vi "Generer_listing.vi"(1 "Listing_entrée":string, 2 "Numéro de programme":u8, 3 "Programme":cluster{"chaîne":string, "Valeur":dbl}[][](array[cluster]) {"Valeur" format="%#.1f"}) -> (0 "Listing_sortie":string)   [LabVIEW 2022 SP3]
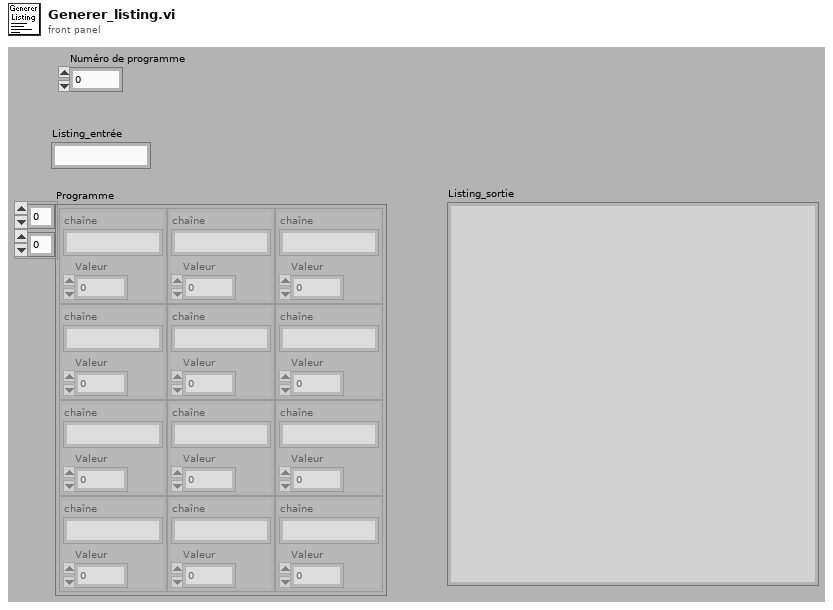
[diagram p1: front panel]
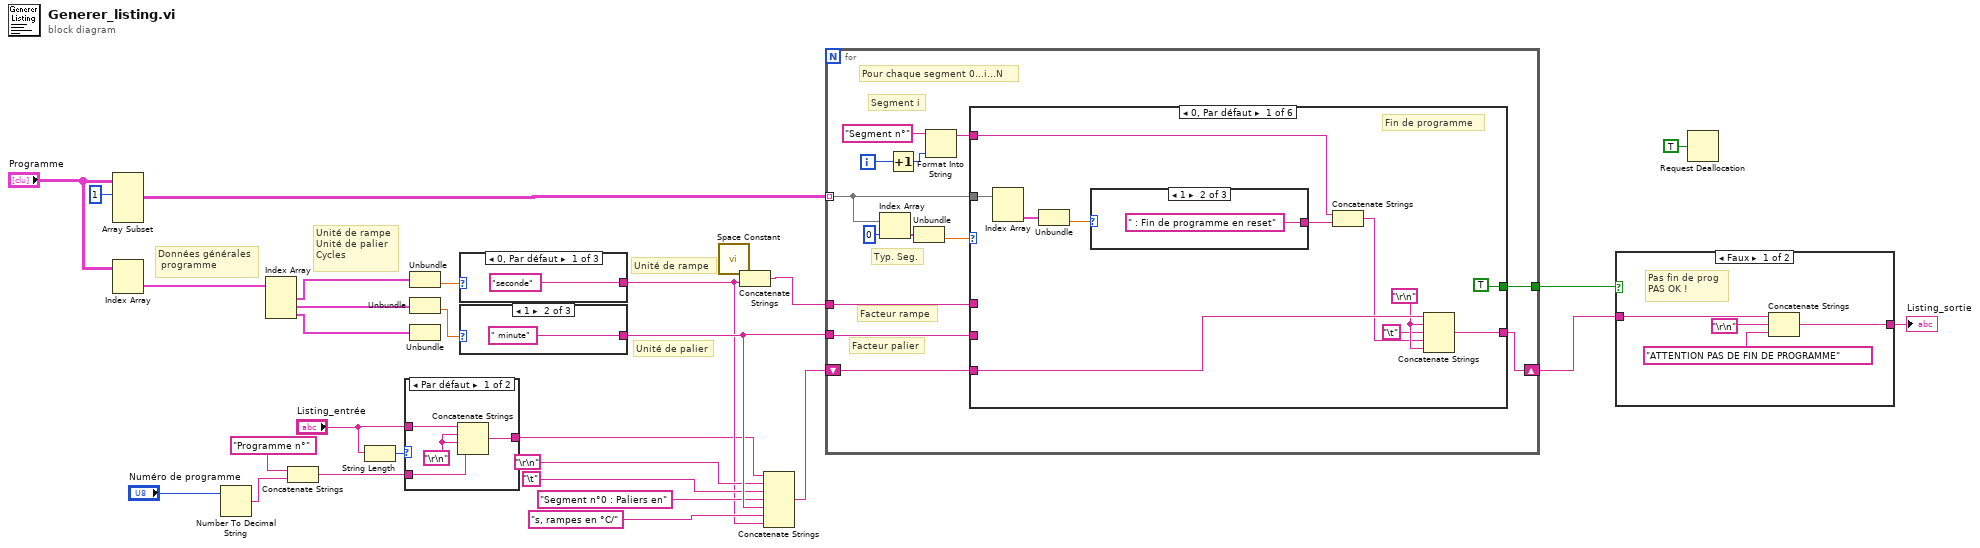
[diagram p0: block diagram]
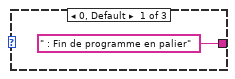
[diagram p3: hidden frame]
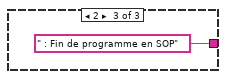
[diagram p4: hidden frame]
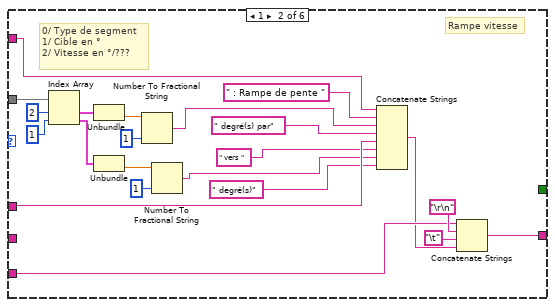
[diagram p5: hidden frame]
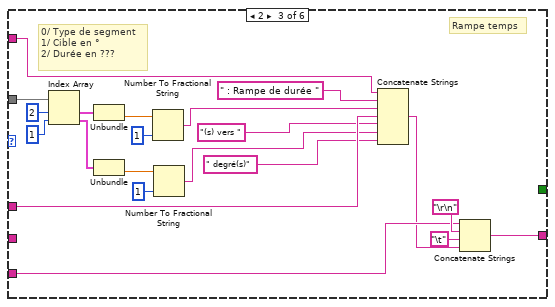
[diagram p6: hidden frame]
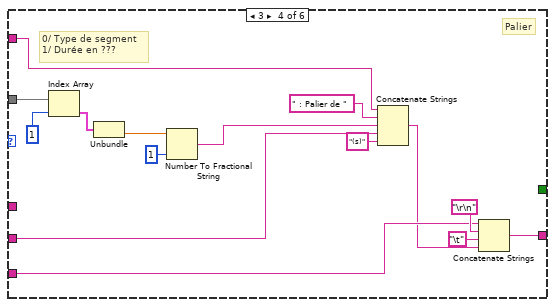
[diagram p7: hidden frame]
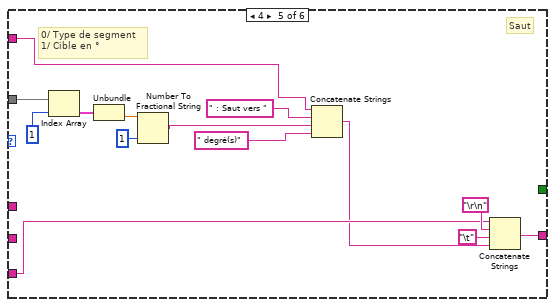
[diagram p8: hidden frame]
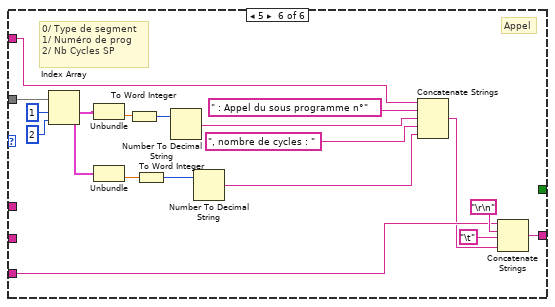
[diagram p9: hidden frame]
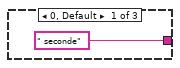
[diagram p11: hidden frame]
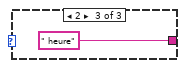
[diagram p12: hidden frame]
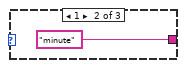
[diagram p13: hidden frame]
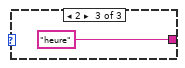
[diagram p14: hidden frame]
diagram:
  # "Unité de rampe"
  # "Unité de palier"
  # "Données générales\n programme"
  # "Unité de rampe\nUnité de palier\nCycles"
  n1 = Array Subset(array="Programme", index (row)=1 ("indice")) -> (w22:cluster{"chaîne":string, "Valeur":dbl}[][])  [unwired: 3 in]
  n2 = Index Array(array="Programme") -> (element=w17:cluster{"chaîne":string, "Valeur":dbl}[])  [unwired: 2 in]
  n3 = Number To Decimal String(number="Numéro de programme") -> (decimal integer string=w26:string)  [unwired: 1 in]
  n4 = Index Array(array=w17) -> (element #1=w16:cluster{"chaîne":string, "Valeur":dbl}, element #2=w15:cluster{"chaîne":string, "Valeur":dbl}, element #3=w14:cluster{"chaîne":string, "Valeur":dbl})  [unwired: 3 in]
  n5 = Concatenate Strings("Programme n°" ("chaîne"), w26) -> (w24:string)
  n6 = String Length(string="Listing_entrée") -> (length=w5:i32)
  n7 = case shown="Par défaut" w5 {
    tunnel: [w33 w34] -> w4
    tunnel: w24 -> [w31 w34]
    tunnel: "Listing_entrée" -> [w30 _]
    frame Default {
      w32 = "\r\n"
      n8 = Concatenate Strings(w30, w32, w32, w31) -> (w33:string)
    }
    frame 0 {
      # "Listing entrée\nvide"
    }
  }
  n9 = Unbundle(w16) -> ("Valeur"=w13:dbl)  [unwired: 1 out]
  n10 = Unbundle(w15) -> ("Valeur"=w12:dbl)  [unwired: 1 out]
  n11 = Unbundle(w14) -> ()  [unwired: 2 out]
  n12 = case shown="0, Par défaut" w13 {
    tunnel: ["seconde" "minute" "heure"] -> w6
    frame 0, Default {
    }
    frame 1 {
    }
    frame 2 {
    }
  }
  n13 = case shown="1" w12 {
    tunnel: [" seconde" " minute" " heure"] -> w20
    frame 0, Default {
    }
    frame 1 {
    }
    frame 2 {
    }
  }
  n14 = call <vilib>:"Space Constant.vi"() -> ("String"=w9:string)
  n15 = Concatenate Strings(w9, w6) -> (w21:string)
  n16 = Concatenate Strings(w4, "\r\n", "\t", "Segment n°0 : Paliers en" ("chaîne"), w20, "s, rampes en °C/" ("chaîne"), w6) -> (w19:string)
  n17 = for {
    tunnel: w22 -> [w51] mode=indexing
    tunnel: w21 -> [w49]
    tunnel: w20 -> [w48]
    shift-right: [w42] -> w2
    shift-left: w19 -> [w50]
    tunnel: [w41] -> w3
    i -> [w46]
    # "Segment i"
    # "Facteur palier"
    # "Pour chaque segment 0...i...N"
    # "Facteur rampe"
    # "Typ. Seg."
    n18 = Index Array(array=w51, index=0 ("indice")) -> (element=w53:cluster{"chaîne":string, "Valeur":dbl})
    n19 = Increment(x=w46) -> (x+1=w44:i32)
    n20 = Unbundle(w53) -> ("Valeur"=w47:dbl)  [unwired: 1 out]
    n21 = Format Into String(initial string="Segment n°" ("chaîne"), w44) -> (resulting string=w43:string)  [unwired: 2 in, 1 out]
    n22 = case shown="0, Par défaut" w47 {
      tunnel: w51 -> [w63 w89 w110 w125 w139 w158]
      tunnel: w49 -> [_ w82 w101 _ _ _]
      tunnel: w48 -> [_ _ _ w118 _ _]
      tunnel: [w61 w78 w103 w121 w135 w151] -> w42
      tunnel: w50 -> [w60 w77 w102 w120 w134 w150]
      tunnel: [TRUE _ _ _ _ _] -> w41
      tunnel: w43 -> [w54 w74 w96 w115 w129 w146]
      frame 0, Default {
        w59 = "\r\n"
        # "Fin de programme"
        n23 = Index Array(array=w63) -> (element #2=w64:cluster{"chaîne":string, "Valeur":dbl})  [unwired: 2 in, 1 out]
        n24 = Unbundle(w64) -> ("Valeur"=w62:dbl)  [unwired: 1 out]
        n25 = case shown="1" w62 {
          tunnel: [" : Fin de programme en palier" " : Fin de programme en reset" " : Fin de programme en SOP"] -> w56
          frame 0, Default {
          }
          frame 1 {
          }
          frame 2 {
          }
        }
        n26 = Concatenate Strings(w54, w56) -> (w55:string)
        n27 = Concatenate Strings(w60, w59, "\t", w55, w59) -> (w61:string)
      }
      frame 1 {
        # "0/ Type de segment\n1/ Cible en °\n2/ Vitesse en °/???"
        # "Rampe vitesse"
        n28 = Index Array(array=w89, index #1=2 ("indice"), index #2=1 ("indice")) -> (element #1=w84:cluster{"chaîne":string, "Valeur":dbl}, element #2=w88:cluster{"chaîne":string, "Valeur":dbl})
        n29 = Unbundle(w84) -> ("Valeur"=w68:dbl)  [unwired: 1 out]
        n30 = Unbundle(w88) -> ("Valeur"=w70:dbl)  [unwired: 1 out]
        n31 = Number To Fractional String(number=w68, precision (6)=i16 1 ("précision (6)")) -> (F-format string=w72:string)  [unwired: 2 in]
        n32 = Number To Fractional String(number=w70, precision (6)=i16 1 ("précision (6)")) -> (F-format string=w69:string)  [unwired: 2 in]
        n33 = Concatenate Strings(w74, " : Rampe de pente " ("chaîne"), w72, " degré(s) par" ("chaîne"), w82, " vers " ("chaîne"), w69, " degré(s)" ("chaîne")) -> (w76:string)
        n34 = Concatenate Strings(w77, "\r\n", "\t", w76) -> (w78:string)
      }
      frame 2 {
        # "0/ Type de segment\n1/ Cible en °\n2/ Durée en ???"
        # "Rampe temps"
        n35 = Index Array(array=w110, index #1=2 ("indice"), index #2=1 ("indice")) -> (element #1=w105:cluster{"chaîne":string, "Valeur":dbl}, element #2=w109:cluster{"chaîne":string, "Valeur":dbl})
        n36 = Unbundle(w105) -> ("Valeur"=w94:dbl)  [unwired: 1 out]
        n37 = Unbundle(w109) -> ("Valeur"=w91:dbl)  [unwired: 1 out]
        n38 = Number To Fractional String(number=w94, precision (6)=i16 1 ("précision (6)")) -> (F-format string=w93:string)  [unwired: 2 in]
        n39 = Number To Fractional String(number=w91, precision (6)=i16 1 ("précision (6)")) -> (F-format string=w90:string)  [unwired: 2 in]
        n40 = Concatenate Strings(w96, " : Rampe de durée " ("chaîne"), w93, w101, "(s) vers " ("chaîne"), w90, " degré(s)" ("chaîne")) -> (w98:string)
        n41 = Concatenate Strings(w102, "\r\n", "\t", w98) -> (w103:string)
      }
      frame 3 {
        # "0/ Type de segment\n1/ Durée en ???"
        # "Palier"
        n42 = Index Array(array=w125, index=1 ("indice")) -> (element=w123:cluster{"chaîne":string, "Valeur":dbl})
        n43 = Unbundle(w123) -> ("Valeur"=w113:dbl)  [unwired: 1 out]
        n44 = Number To Fractional String(number=w113, precision (6)=i16 1 ("précision (6)")) -> (F-format string=w112:string)  [unwired: 2 in]
        n45 = Concatenate Strings(w115, " : Palier de " ("chaîne"), w112, w118, "(s)" ("chaîne")) -> (w117:string)
        n46 = Concatenate Strings(w120, "\r\n", "\t", w117) -> (w121:string)
      }
      frame 4 {
        # "0/ Type de segment\n1/ Cible en °"
        # "Saut"
        n47 = Index Array(array=w139, index=1 ("indice")) -> (element=w137:cluster{"chaîne":string, "Valeur":dbl})
        n48 = Unbundle(w137) -> ("Valeur"=w127:dbl)  [unwired: 1 out]
        n49 = Number To Fractional String(number=w127, precision (6)=i16 1 ("précision (6)")) -> (F-format string=w126:string)  [unwired: 2 in]
        n50 = Concatenate Strings(w129, " : Saut vers " ("chaîne"), w126, " degré(s)" ("chaîne")) -> (w131:string)
        n51 = Concatenate Strings(w134, "\r\n", "\t", w131) -> (w135:string)
      }
      frame 5 {
        # "0/ Type de segment\n1/ Numéro de prog\n2/ Nb Cycles SP"
        # "Appel"
        n52 = Index Array(array=w158, index #1=1 ("indice"), index #2=2 ("indice")) -> (element #1=w153:cluster{"chaîne":string, "Valeur":dbl}, element #2=w157:cluster{"chaîne":string, "Valeur":dbl})
        n53 = Unbundle(w153) -> ("Valeur"=w143:dbl)  [unwired: 1 out]
        n54 = Unbundle(w157) -> ("Valeur"=w141:dbl)  [unwired: 1 out]
        n55 = To Word Integer(number=w143) -> (16bit integer=w142:i16)
        n56 = To Word Integer(number=w141) -> (16bit integer=w140:i16)
        n57 = Number To Decimal String(number=w142) -> (decimal integer string=w145:string)  [unwired: 1 in]
        n58 = Number To Decimal String(number=w140) -> (decimal integer string=w144:string)  [unwired: 1 in]
        n59 = Concatenate Strings(w146, " : Appel du sous programme n°" ("chaîne"), w145, ", nombre de cycles : " ("chaîne"), w144) -> (w148:string)
        n60 = Concatenate Strings(w150, "\r\n", "\t", w148) -> (w151:string)
      }
    }
  }
  n61 = case shown="Faux" w3 {
    tunnel: w2 -> [w161 w163]
    tunnel: [w162 w163] -> w1
    frame False {
      # "Pas fin de prog\nPAS OK !"
      n62 = Concatenate Strings(w161, "\r\n", "ATTENTION PAS DE FIN DE PROGRAMME" ("chaîne")) -> (w162:string)
    }
    frame True {
      # "Fin de programme\nOK !"
    }
  }
  "Listing_sortie" <- w1
  n63 = Request Deallocation(TRUE ("flag")) -> ()
